vi "Dependencies.vi"() -> (3 "Dependencies":T1)   [LabVIEW 2024]
uses:
  Provider/Provider.lvclass
  Dependencies.ctl
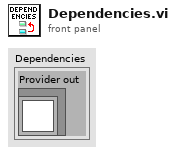
[diagram p1: front panel]
types:
  T1 = typedef "Dependencies.ctl" = cluster{"Provider out":refnum<class "Provider.lvclass">}
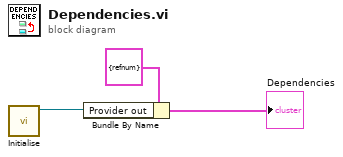
[diagram p0: block diagram]
diagram:
  n1 = call "Initialise.vi"() -> ("Provider out"=w3:refnum<class "Provider.lvclass">)  [unwired: 9 in, 2 out]
  n2 = Bundle By Name(cluster=T1 {"Provider out"=refnum} ("Dependencies"), "Provider out"=w3) -> (→"Dependencies":T1)
